vi "ContextHelp_PopUp.vi"() -> ()   [LabVIEW 2020]
uses:
  <resource>/Framework/Providers/Open_GDS/UML/ContextHelp/ContextHelp_EventType.ctl
  <resource>/Framework/Providers/Open_GDS/UML/ContextHelp/ContextHelp_ShowType.ctl
  <vilib>/event_ctls.llb/eventvkey.ctl
panel:
  in  "CallerRef":refnum<vi>
  in  "OccSync":refnum<k4>
  in  "Event":T1
  out "new picture":picture
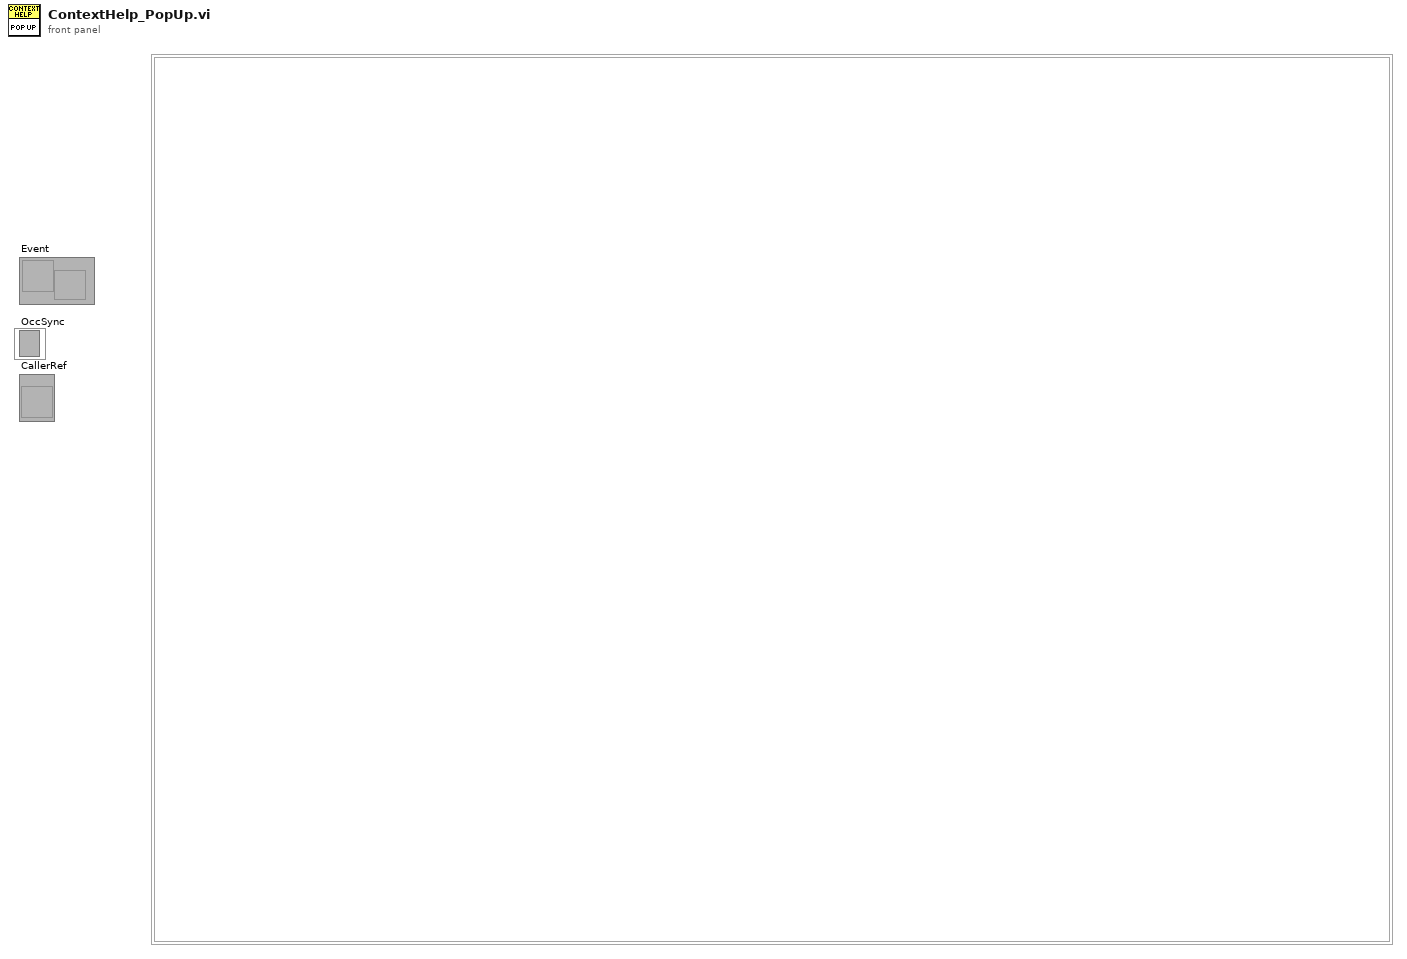
[diagram p1: front panel]
types:
  T1 = typedef "ContextHelp_EventType.ctl" = refnum<user-event>
  T2 = typedef "ContextHelp_ShowType.ctl" = cluster{"Header":string, "Picture":picture, "Text":string}
  T3 = cluster{"VIs":refnum<vi>[], "ViPathes":path[], "VI":i32, "Show":T2, "Win":cluster{"left":i16, "top":i16, "right":i16, "bottom":i16}, "LastViRef":refnum<vi>}
  T4 = enum32{"Custom", "Standard", "Using Panel", "Using SubVI", "Complete"}
  T5 = enum16{"SetPopUpEventTask", "GetStatus", "SetOpenState"}
  T6 = cluster{"left":i16, "top":i16, "right":i16, "bottom":i16}
  T7 = typedef "eventvkey.ctl" = enum16{"ASCII", "Enter", "Return", "Shift", "Ctrl", "Alt", "Cmd", "Opt", "Caps", "NumLock", "Clear", "Break", "Up", "Down", "Left", "Right", "Insert", "Delete", "Home", "End", "PageUp", "PageDown", "Escape", "Help", "Pause", "ScrollLock", "F1", "F2", "F3", "F4", "F5", "F6", "F7", "F8", "F9", "F10", "F11", "F12", "F13", "F14", "F15", "F16", "F17", "F18", "F19", "F20", "F21", "F22", "F23", "F24", "Play", "VolumeUp", "VolumeDown", "Mute", "Two Byte Char"}
  T8 = typedef "Librarian File Info Out.ctl" = cluster{"creation date":u32, "last mod date":u32, "type":string, "creator":string, "LV version":i32, "size":i32, "top level":bool}
  T9 = typedef "imagedata.ctl" = cluster{"image type":i32, "image depth":i32, "image":u8[], "mask":u8[], "colors":u32[], "Rectangle":cluster{"left":i16, "top":i16, "right":i16, "bottom":i16}}
  T10 = cluster{"Font Name:":string, "Size":i16, "Strikeout?":bool, "Italic?":bool, "Underline?":bool, "Outline?":bool, "Shadow?":bool, "Bold?":bool}
  T11 = enum16{"User-specified Font", "Application Font", "System Font", "Dialog Font"}
  T12 = typedef "LVRectTypeDef.ctl" = cluster{"Left":i16, "Top":i16, "Right":i16, "Bottom":i16}
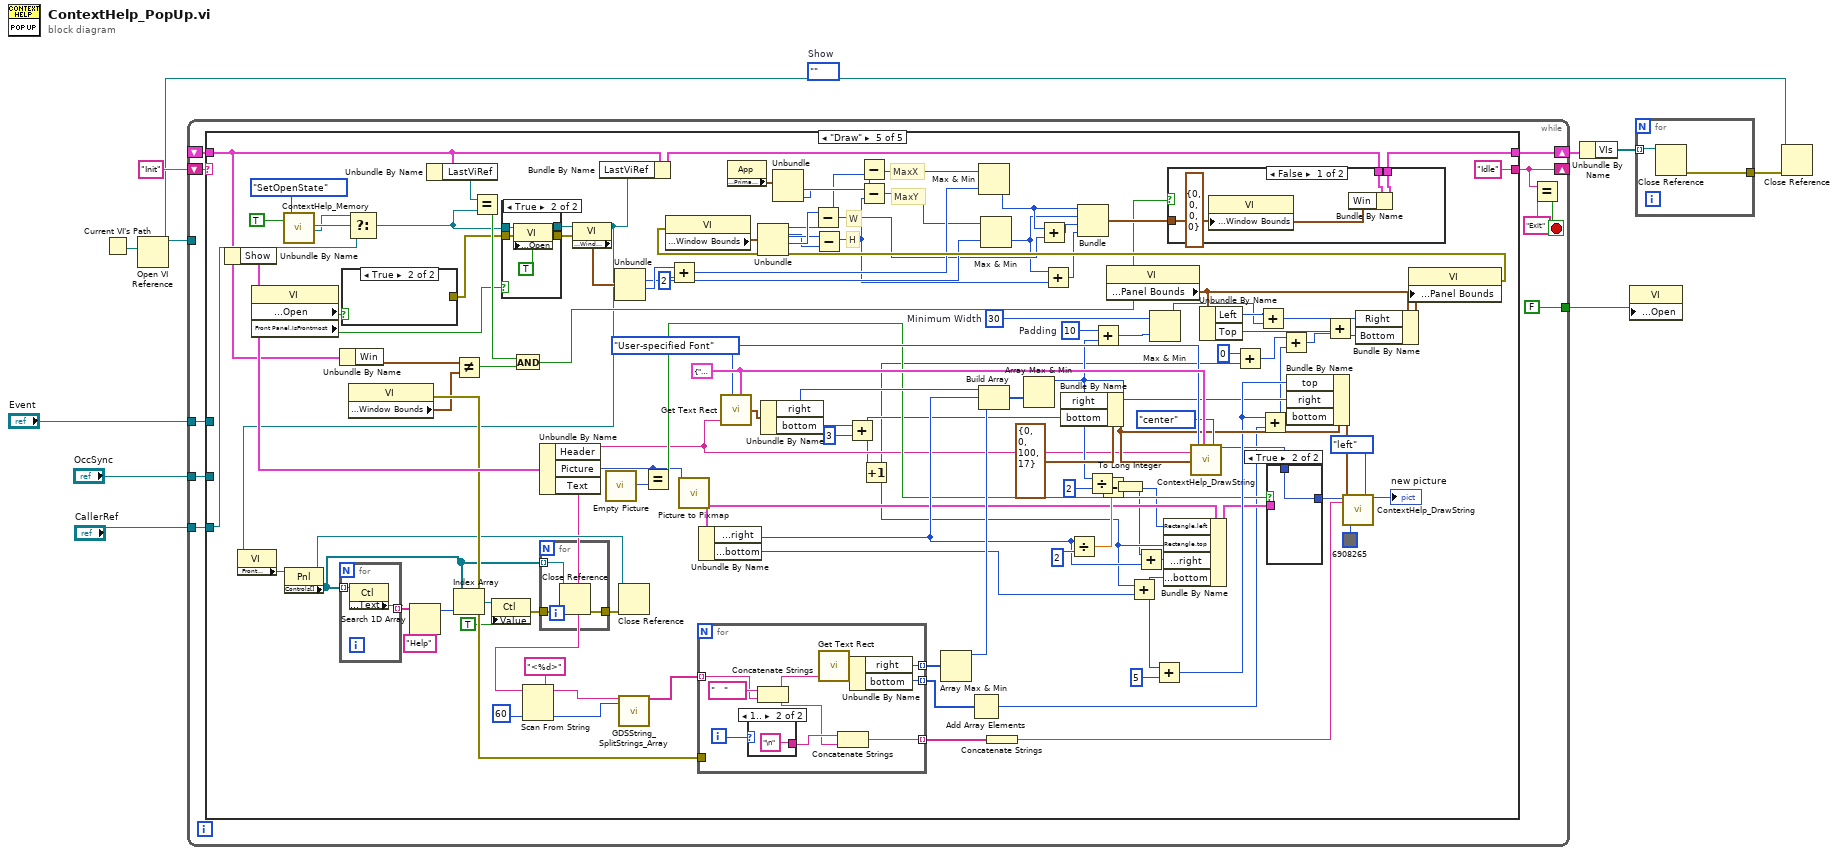
[diagram p0: block diagram]
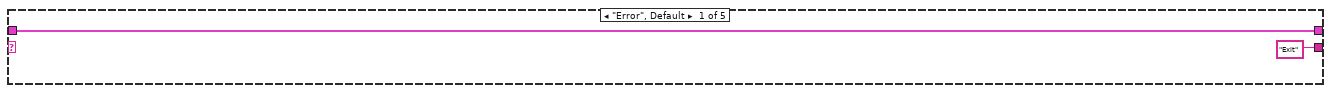
[diagram p2: hidden frame]
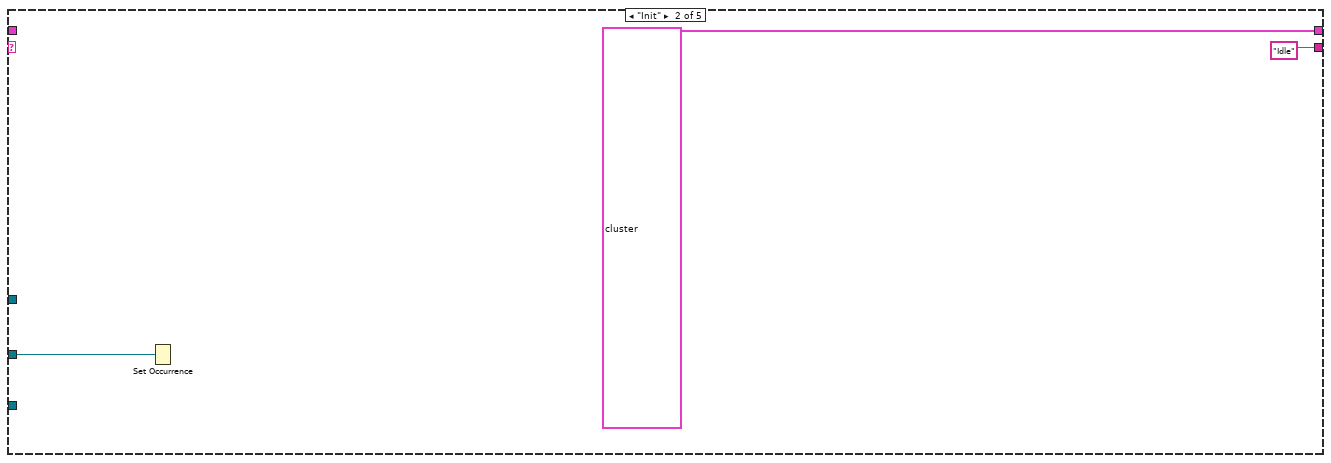
[diagram p3: hidden frame]
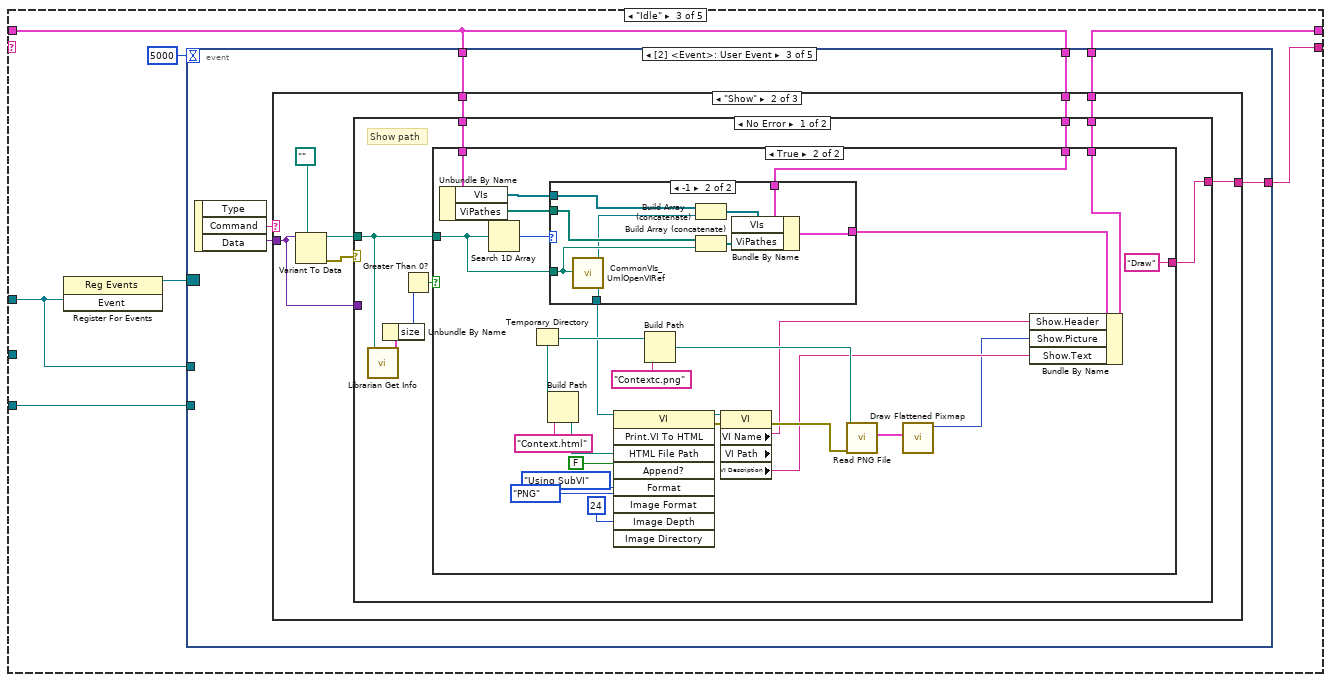
[diagram p4: hidden frame]
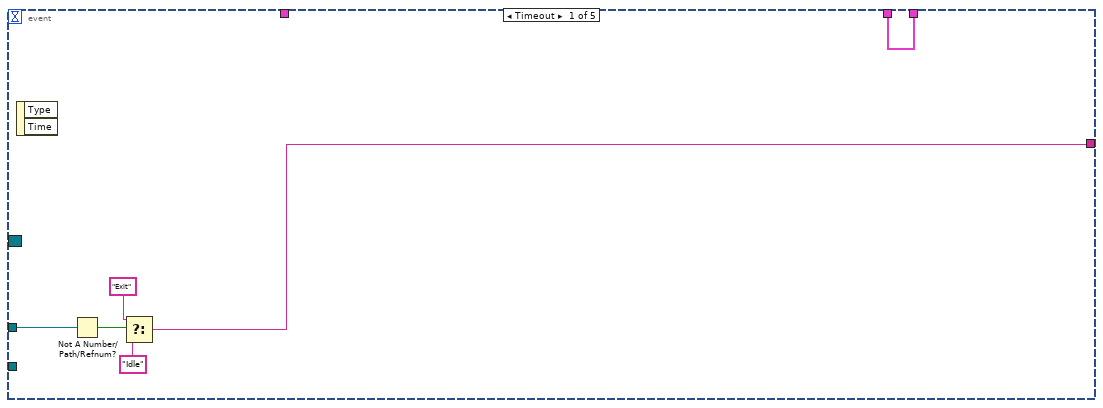
[diagram p5: hidden frame]
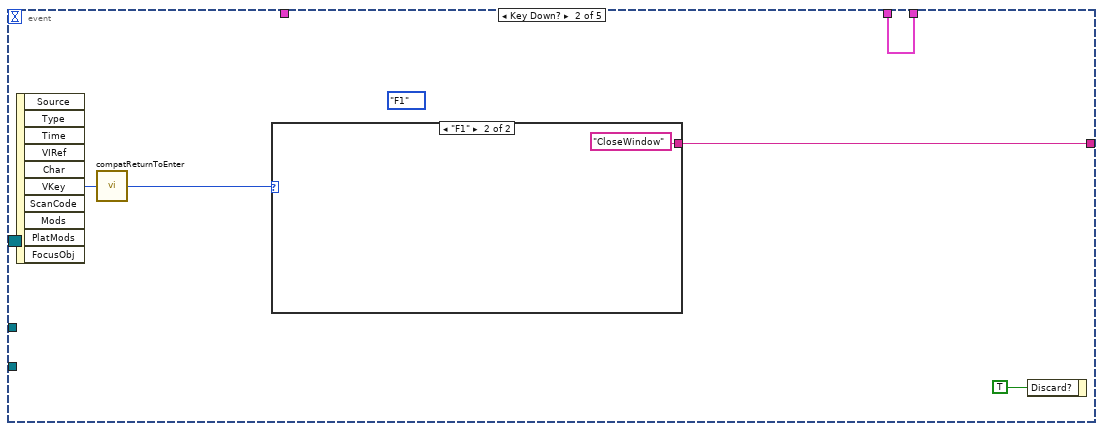
[diagram p6: hidden frame]
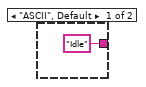
[diagram p7: hidden frame]
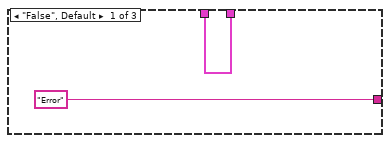
[diagram p8: hidden frame]
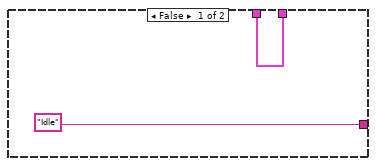
[diagram p9: hidden frame]
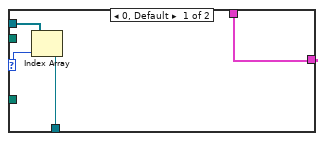
[diagram p10: hidden frame]
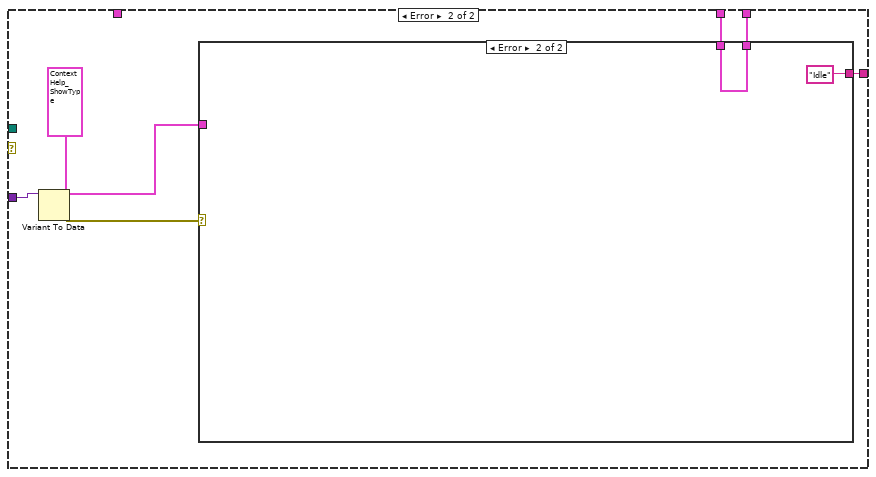
[diagram p11: hidden frame]
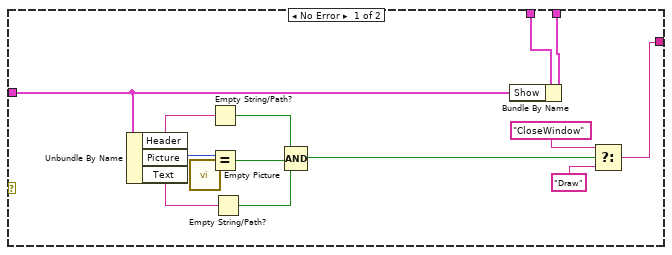
[diagram p12: hidden frame]
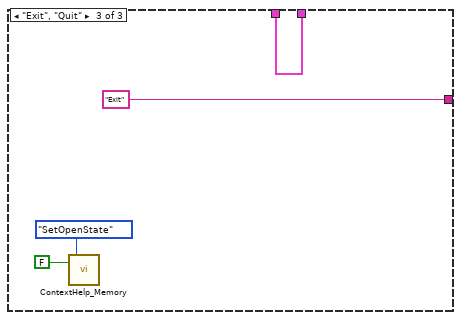
[diagram p13: hidden frame]
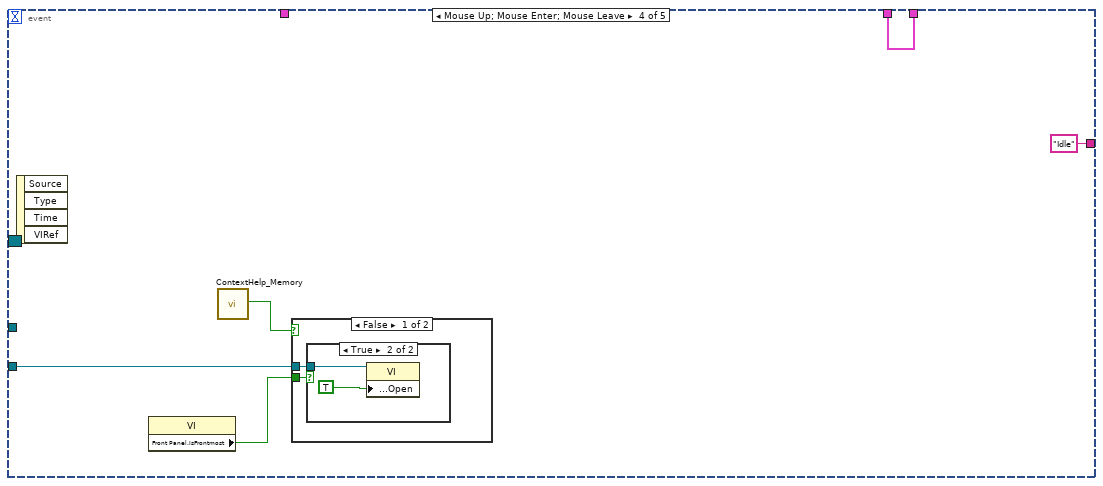
[diagram p14: hidden frame]
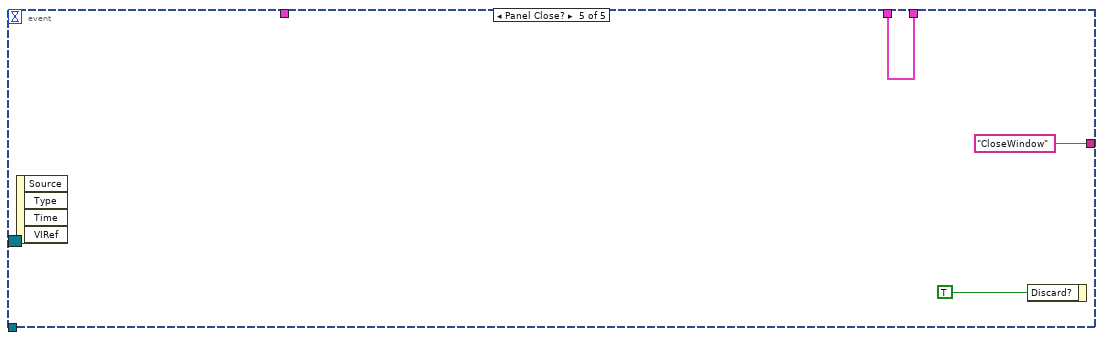
[diagram p17: hidden frame]
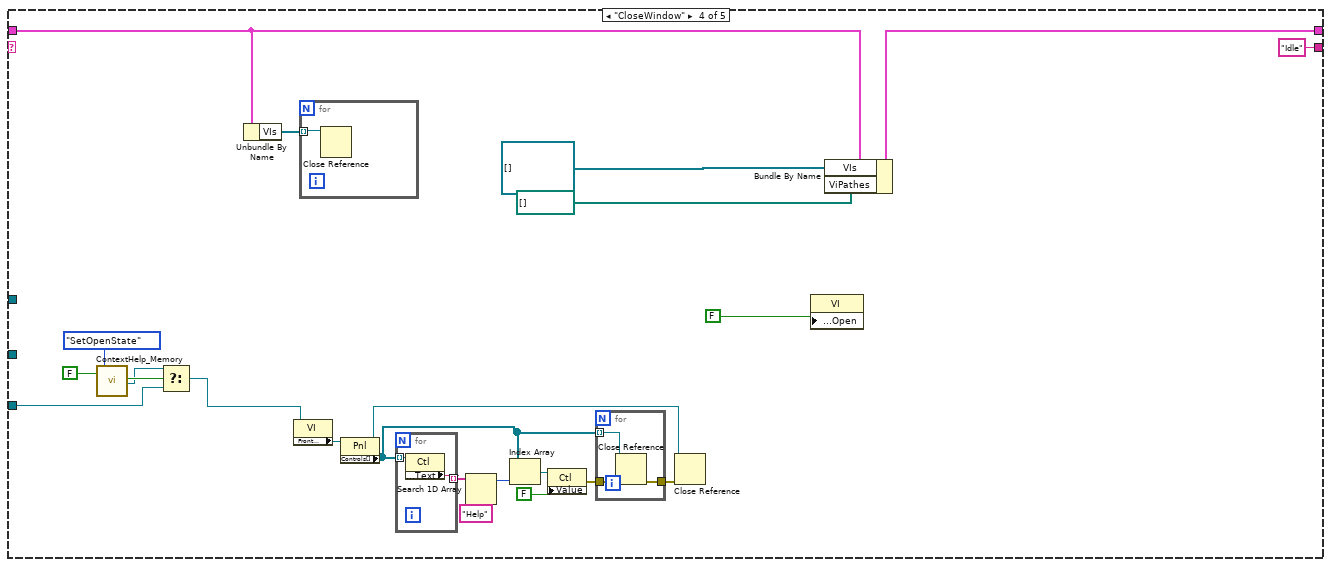
[diagram p18: hidden frame]
diagram:
  (unwired) enum16{"ClassDescription", ""}.""  # Show
  n1 = Current VI's Path() -> (path=w6:path)
  n2 = Open VI Reference(vi path=w6) -> (vi reference=w4:refnum<vi>)  [unwired: 2 in, 4 out]
  n3 = while {
    shift-right: [w19] -> _
    shift-left: "Init" -> [w20]
    shift-right: [w16] -> w8
    shift-left: _ -> [w15]
    tunnel: "Event" -> [w14]
    tunnel: w4 -> [_]
    tunnel: "OccSync" -> [w13]
    tunnel: [FALSE ("Front Panel Window:Open")] -> w2
    tunnel: "CallerRef" -> [w11]
    stop <- w17 stop-if-true
    n4 = case shown="\"Draw\"" w20 {
      tunnel: ["Exit" "Idle" w31 "Idle" "Idle"] -> w19
      tunnel: [w21 T3 {"VIs"=[], "ViPathes"=[], "VI"=0, "Show"={"Header"="", "Picture"=bytes[0], "Text"=""}, "Win"={"left"=0, "top"=0, "right"=0, "bottom"=0}, "LastViRef"=refnum} w30 w156 w210] -> w16
      tunnel: w15 -> [w21 _ w29 w157 w208]
      tunnel: w14 -> [_ _ w27 _ _]
      tunnel: w13 -> [_ w23 _ _ _]
      tunnel: w11 -> [_ _ w26 w150 w236]
      frame "Error", Default {
      }
      frame "Init" {
        n5 = Set Occurrence(w23) -> ()
      }
      frame "Idle" {
        n6 = register-events(w27) -> (reference out=w32:refnum<event-registration>)  [unwired: 2 in, 1 out]
        n7 = event shown="[2] <Event>: User Event" {
          selector: w32 -> [_ _ _ _ _]
          dyn-events: _ -> [_ _ _ _ _]
          timeout: 5000 -> [_ _ _ _ _]
          tunnel: [w34 w41 w50 "Idle" "CloseWindow"] -> w31
          tunnel: w29 -> [w38 w43 w49 w141 w146]
          tunnel: [w38 w43 w48 w141 w146] -> w30
          tunnel: w29 -> [_ _ w46 _ _]
          tunnel: w27 -> [w37 _ _ _ _]
          tunnel: w26 -> [_ _ _ w139 _]
          event Timeout {
            n8 = event-data() -> ()  [unwired: 3 out]
            n9 = Not A Number/Path/Refnum?(number/path/refnum=w37) -> (NaN/Path/Refnum?=w36:bool)
            n10 = Select(t="Exit", s=w36, f="Idle") -> (s? t:f=w34:string)
          }
          event Key Down? {
            (unwired) eventvkey."F1" ("VKey")
            n11 = event-data() -> ("VKey"=w39:T7)  [unwired: 10 out]
            n12 = call <vilib>:"compatReturnToEnter.vi"("VKey"=w39) -> ("VKey"=w42:T7)
            n13 = case shown="\"F1\"" w42 {
              tunnel: ["Idle" "CloseWindow"] -> w41
              frame "ASCII", Default {
              }
              frame "F1" {
              }
            }
            n14 = event-data("Discard?"=TRUE) -> ()  [unwired: 1 in, 1 out]
          }
          event User Event {
            n15 = event-data() -> ("Command"=w51:string, "Data"=w47:variant)  [unwired: 2 out]
            n16 = case shown="\"Show\"" w51 {
              tunnel: ["Error" w56 "Exit"] -> w50
              tunnel: w49 -> [w53 w59 w135]
              tunnel: [w53 w58 w135] -> w48
              tunnel: w47 -> [_ w54 _]
              tunnel: w46 -> [_ w60 _]
              frame "False", Default {
              }
              frame "Show" {
                n17 = Variant To Data(type=path "", Variant=w54) -> (data=w57:path, error out=w55:errorcluster)  [unwired: 1 in]
                n18 = case shown="No Error" w55 {
                  tunnel: w60 -> [w69 _]
                  tunnel: w59 -> [w68 w115]
                  tunnel: [w67 w114] -> w58
                  tunnel: w57 -> [w65 _]
                  tunnel: [w66 w111] -> w56
                  tunnel: w54 -> [_ w116]
                  frame No Error {
                    # "Show path"
                    n19 = call <vilib>:"Librarian Get Info.vi"("path"=w65) -> ("file information"=w64:T8)  [unwired: 1 in, 9 out]
                    n20 = Unbundle By Name(w64) -> ("size"=w63:i32)
                    n21 = Greater Than 0?(x=w63) -> (x > 0?=w62:bool)
                    n22 = case shown="True" w62 {
                      tunnel: w69 -> [_ w97]
                      tunnel: w68 -> [w71 w95]
                      tunnel: [w71 w90] -> w67
                      tunnel: w65 -> [_ w92]
                      tunnel: ["Idle" "Draw"] -> w66
                      frame False {
                      }
                      frame True {
                        n23 = Unbundle By Name(w97) -> ("VIs"=w94:refnum<vi>[], "ViPathes"=w93:path[])
                        n24 = Search 1D Array(1D array=w93, element=w92) -> (index of element=w96:i32)  [unwired: 1 out]
                        n25 = Temporary Directory() -> (w81:path)
                        n26 = Build Path(base path=w81, name or relative path="Context.html") -> (appended path=w79:path)
                        n27 = case shown="-1" w96 {
                          selector: w96 -> [w101 _]
                          tunnel: w92 -> [_ w103]
                          tunnel: w95 -> [w98 w109]
                          tunnel: w94 -> [w100 w108]
                          tunnel: w93 -> [_ w105]
                          tunnel: [w98 w104] -> w89
                          tunnel: [w99 w102] -> w76
                          frame 0, Default {
                            n28 = Index Array(array=w100, index=w101) -> (element=w99:refnum<vi>)
                          }
                          frame -1 {
                            n29 = call <resource>:"CommonVIs_UmlOpenVIRef.vi"("ViPath/ViName"=w103) -> ("vi reference"=w102:refnum<vi>)  [unwired: 3 in, 7 out]
                            n30 = Build Array (concatenate)(w108, w102) -> (w107:refnum<vi>[])
                            n31 = Build Array (concatenate)(w105, w103) -> (w106:path[])
                            n32 = Bundle By Name(cluster=w109, "VIs"=w107, "ViPathes"=w106) -> (w104:T3)
                          }
                        }
                        n33 = invoke class="VI" method="Print.VI To HTML"(reference=w76, "HTML File Path"=w79, "Append?"=FALSE, "Format"=T4."Using SubVI", "Image Format"=enum32{"PNG", "JPEG", "GIF"}."PNG", "Image Depth"=24) -> (reference out=w86:refnum<vi>, error out=w85:errorcluster)  [unwired: 3 in, 7 out]
                        n34 = Build Path(base path=w81, name or relative path="Contextc.png" ("HTML File Path")) -> (appended path=w78:path)
                        n35 = property class="VI" props=["VI Name", "VI Path", "VI Description"](reference=w86, error in=w85) -> (error out=w84:errorcluster, "VI Name"=w75:string, "VI Description"=w74:string)  [unwired: 2 out]
                        n36 = call <vilib>:"Read PNG File.vi"("error in (no error)"=w84, "path to PNG file"=w78) -> ("image data"=w73:T9)  [unwired: 9 out]
                        n37 = call <vilib>:"Draw Flattened Pixmap.vi"("image data"=w73) -> ("new picture"=w72:picture)  [unwired: 1 in, 7 out]
                        n38 = Bundle By Name(cluster=w89, "Show.Header"=w75, "Show.Picture"=w72, "Show.Text"=w74) -> (w90:T3)
                      }
                    }
                  }
                  frame Error {
                    n39 = Variant To Data(type=T2 {"Header"="", "Picture"=bytes[0], "Text"=""} ("output cluster"), Variant=w116) -> (data=w113:T2, error out=w112:errorcluster)  [unwired: 1 in]
                    n40 = case shown="Error" w112 {
                      tunnel: w115 -> [w130 w131]
                      tunnel: [w129 w131] -> w114
                      tunnel: w113 -> [w128 _]
                      tunnel: [w119 "Idle"] -> w111
                      frame No Error {
                        n41 = Unbundle By Name(w128) -> ("Header"=w124:string, "Picture"=w127:picture, "Text"=w125:string)
                        n42 = call "Empty Picture"() -> ("empty picture"=w126:picture)
                        n43 = Empty String/Path?(string/path=w124) -> (empty?=w123:bool)
                        n44 = Equal?(x=w127, y=w126) -> (x = y?=w122:bool)
                        n45 = Empty String/Path?(string/path=w125) -> (empty?=w121:bool)
                        n46 = Compound Arithmetic op=AND(w123, w122, w121) -> (w117:bool)
                        n47 = Bundle By Name(cluster=w130, "Show"=w128) -> (w129:T3)
                        n48 = Select(t="CloseWindow", s=w117, f="Draw") -> (s? t:f=w119:string)
                      }
                      frame Error {
                      }
                    }
                  }
                }
              }
              frame "Exit", "Quit" {
                n49 = call <resource>:"ContextHelp_Memory.vi"("State"=FALSE ("OpenState"), "Actio(GetStatus)n"=T5."SetOpenState") -> ()  [unwired: 2 in, 16 out]
              }
            }
          }
          event Mouse Up; Mouse Enter; Mouse Leave {
            n50 = event-data() -> ()  [unwired: 5 out]
            n51 = property class="VI"() -> ("Front Panel.IsFrontmost"=w137:bool)  [unwired: 2 in, 2 out]
            n52 = call <resource>:"ContextHelp_Memory.vi"() -> ("DialogCaller"=w138:bool)  [unwired: 4 in, 15 out]
            n53 = case shown="False" w138 {
              tunnel: w139 -> [w143 _]
              tunnel: w137 -> [w142 _]
              frame False {
                n54 = case shown="True" w142 {
                  tunnel: w143 -> [_ w145]
                  frame False {
                  }
                  frame True {
                    n55 = property class="VI"(reference=w145, "Front Panel Window:Open"=TRUE ("Front Panel Window:Is Frontmost")) -> ()  [unwired: 1 in, 2 out]
                  }
                }
              }
              frame True {
              }
            }
          }
          event Panel Close? {
            n56 = event-data() -> ()  [unwired: 5 out]
            n57 = event-data("Discard?"=TRUE) -> ()  [unwired: 1 in, 1 out]
          }
        }
      }
      frame "CloseWindow" {
        n58 = call <resource>:"ContextHelp_Memory.vi"("State"=FALSE ("OpenState"), "Actio(GetStatus)n"=T5."SetOpenState") -> ("DialogCaller"=w152:bool, "DialogRef"=w151:refnum<vi>)  [unwired: 2 in, 14 out]
        n59 = Select(t=w151, s=w152, f=w150) -> (s? t:f=w149:refnum<vi>)
        n60 = Unbundle By Name(w157) -> ("VIs"=w170:refnum<vi>[])
        n61 = property class="VI"(reference=w149) -> ("Front Panel"=w167:refnum<vi>)  [unwired: 1 in, 2 out]
        n62 = for {
          tunnel: w170 -> [w177] mode=indexing
          n63 = Close Reference(reference=w177) -> ()  [unwired: 1 in, 1 out]
        }
        n64 = property class="Pnl"(reference=w167) -> (reference out=w158:refnum<vi>, "Controls[]"=w160:refnum<vi>[])  [unwired: 1 in, 1 out]
        n65 = for {
          tunnel: w160 -> [w176] mode=indexing
          tunnel: [w175] -> w166 mode=indexing
          n66 = property class="Ctl"(reference=w176) -> ("Label.Text"=w175:string)  [unwired: 1 in, 2 out]
        }
        n67 = Search 1D Array(1D array=w166, element="Help") -> (index of element=w164:i32)  [unwired: 1 out]
        n68 = Index Array(array=w160, index=w164) -> (element=w163:refnum<vi>)
        n69 = property class="Ctl"(reference=w163, "Value"=FALSE ("Discard?")) -> (error out=w161:errorcluster)  [unwired: 1 in, 1 out]
        n70 = for {
          tunnel: w161 -> [w174]
          tunnel: w160 -> [w173] mode=indexing
          tunnel: [w172] -> w159
          n71 = Close Reference(reference=w173, error in (no error)=w174) -> (error out=w172:errorcluster)
        }
        n72 = Close Reference(reference=w158, error in (no error)=w159) -> ()  [unwired: 1 out]
        n73 = property class="VI"("Front Panel Window:Open"=FALSE) -> ()  [unwired: 2 in, 2 out]
        n74 = Bundle By Name(cluster=w157, "VIs"=refnum<vi>[] [], "ViPathes"=path[] []) -> (w156:T3)
      }
      frame "Draw" {
        w178 = i16 30  # Minimum Width
        w292 = T10 {"Font Name:"="Ariel", "Size"=14, "Strikeout?"=FALSE, "Italic?"=FALSE, "Underline?"=FALSE, "Outline?"=FALSE, "Shadow?"=FALSE, "Bold?"=TRUE} ("[user-specified font]")
        w247 = i16 10  # Padding
        w291 = T11."User-specified Font" ("desired font(Application)")
        # "MaxX"
        # "MaxY"
        # "H"
        # "W"
        n75 = Unbundle By Name(w208) -> ("Show"=w256:T2)
        n76 = property class="VI"() -> ("Front Panel Window:Open"=w241:bool, "Front Panel.IsFrontmost"=w181:bool)  [unwired: 2 in, 2 out]
        n77 = call <resource>:"ContextHelp_Memory.vi"("State"=TRUE ("OpenState"), "Actio(GetStatus)n"=T5."SetOpenState") -> ("DialogCaller"=w237:bool, "DialogRef"=w235:refnum<vi>)  [unwired: 2 in, 14 out]
        n78 = Unbundle By Name(w208) -> ("Win"=w206:T6)
        n79 = case shown="True" w241 {
          tunnel: [w314 _] -> w184
          frame False {
            n80 = property class="VI"("Front Panel Window:Open"=TRUE) -> (error out=w314:errorcluster)  [unwired: 2 in, 1 out]
          }
          frame True {
          }
        }
        n81 = Select(t=w235, s=w237, f=w236) -> (s? t:f=w185:refnum<vi>)
        n82 = property class="VI"() -> (error out=w211:errorcluster, "Front Panel Window:Window Bounds"=w207:T12)  [unwired: 2 in, 1 out]
        n83 = Unbundle By Name(w208) -> ("LastViRef"=w205:refnum<vi>)
        n84 = Not Equal?(x=w206, y=w207) -> (x != y?=w204:bool)
        n85 = Equal?(x=w205, y=w185) -> (x = y?=w186:bool)
        n86 = case shown="True" w181 {
          tunnel: w185 -> [w299 w304]
          tunnel: w184 -> [w298 w303]
          tunnel: [w299 w302] -> w183
          tunnel: [w298 w301] -> w182
          frame False {
          }
          frame True {
            n87 = property class="VI"(reference=w304, error in=w303, "Front Panel Window:Open"=TRUE) -> (reference out=w302:refnum<vi>, error out=w301:errorcluster)
          }
        }
        n88 = And(x=w186, y=w204) -> (x .and. y?=w203:bool)
        n89 = Unbundle By Name(w256) -> ("Header"=w251:string, "Picture"=w253:picture, "Text"=w187:string)
        n90 = Scan From String(format string="<%d>" ("regular expression"), input string=w187, default 1=60 ("Max string length")) -> (remaining string=w188:string, output 1=w189:i32)  [unwired: 2 in, 2 out]
        n91 = property class="VI"(reference=w183, error in=w182) -> (reference out=w192:refnum<vi>, "Front Panel Window:Window Bounds"=w225:T12)  [unwired: 1 out]
        n92 = property class="VI"(reference=w192) -> ("Front Panel"=w202:refnum<vi>)  [unwired: 1 in, 2 out]
        n93 = property class="Pnl"(reference=w202) -> (reference out=w193:refnum<vi>, "Controls[]"=w195:refnum<vi>[])  [unwired: 1 in, 1 out]
        n94 = for {
          tunnel: w195 -> [w309] mode=indexing
          tunnel: [w308] -> w201 mode=indexing
          n95 = property class="Ctl"(reference=w309) -> ("Label.Text"=w308:string)  [unwired: 1 in, 2 out]
        }
        n96 = Search 1D Array(1D array=w201, element="Help") -> (index of element=w199:i32)  [unwired: 1 out]
        n97 = Index Array(array=w195, index=w199) -> (element=w198:refnum<vi>)
        n98 = property class="Ctl"(reference=w198, "Value"=TRUE ("Discard?")) -> (error out=w196:errorcluster)  [unwired: 1 in, 1 out]
        n99 = for {
          tunnel: w196 -> [w307]
          tunnel: w195 -> [w306] mode=indexing
          tunnel: [w305] -> w194
          n100 = Close Reference(reference=w306, error in (no error)=w307) -> (error out=w305:errorcluster)
        }
        n101 = Bundle By Name(cluster=w208, "LastViRef"=w192) -> (w209:T3)
        n102 = call "Empty Picture"() -> ("empty picture"=w255:picture)
        n103 = Unbundle(w225) -> ("Top"=w218:i16, "Right"=w224:i16)  [unwired: 2 out]
        n104 = Close Reference(reference=w193, error in (no error)=w194) -> ()  [unwired: 1 out]
        n105 = call <resource>:"GDSString_SplitStrings_Array.vi"("string"=w188, "Max string length"=w189) -> ("Array"=w259:string[])  [unwired: 17 out]
        n106 = Equal?(x=w253, y=w255) -> (x = y?=w254:bool)
        n107 = Add(x=w224, y=i16 2) -> (x+y=w220:i16)
        n108 = call <vilib>:"Picture to Pixmap.vi"("picture"=w253) -> ("image data"=w252:T9)  [unwired: 3 in, 7 out]
        n109 = for {
          tunnel: w259 -> [w324] mode=indexing
          tunnel: [w327] -> w296 mode=indexing
          tunnel: [w326] -> w243 mode=indexing
          tunnel: [w323] -> w258 mode=indexing
          tunnel: w211 -> [_]
          i -> [w322]
          n110 = case shown="1.." w322 {
            tunnel: ["" "\n"] -> w321
            frame 0, Default {
            }
            frame 1.. {
            }
          }
          n111 = Concatenate Strings("   " ("replace string (\"\")"), w324) -> (w320:string)
          n112 = call <vilib>:"Get Text Rect.vi"("text"=w320) -> ("rect"=w328:T6)  [unwired: 5 in, 3 out]
          n113 = Concatenate Strings(w321, w320) -> (w323:string)
          n114 = Unbundle By Name(w328) -> ("right"=w327:i16, "bottom"=w326:i16)
        }
        n115 = Unbundle By Name(w252) -> ("Rectangle.right"=w281:i16, "Rectangle.bottom"=w282:i16)
        n116 = call <vilib>:"Get Text Rect.vi"("desired font(Application)"=w291, "text"=w251, "[user-specified font]"=w292) -> ("rect"=w297:T6)  [unwired: 3 in, 3 out]
        n117 = property class="App"() -> ("Display:Primary Workspace"=w228:T12)  [unwired: 2 in, 2 out]
        n118 = Unbundle By Name(w297) -> ("right"=w295:i16, "bottom"=w250:i16)
        n119 = Unbundle(w228) -> ("Right"=w227:i16, "Bottom"=w226:i16)  [unwired: 2 out]
        n120 = Add(x=w250, y=i16 3) -> (x+y=w248:i16)
        n121 = Increment(x=w248) -> (x+1=w244:i16)
        n122 = Array Max & Min(array=w296) -> (max value=w294:i16)  [unwired: 3 out]
        n123 = Add Array Elements(numeric array=w243) -> (sum=w242:i16)
        n124 = Build Array(w295, w281, w294) -> (w293:i16[])
        n125 = Concatenate Strings(w258) -> (w257:string)
        n126 = Array Max & Min(array=w293) -> (max value=w267:i16)  [unwired: 3 out]
        n127 = Bundle By Name(cluster=T6 {"left"=0, "top"=0, "right"=100, "bottom"=17} ("rect"), "right"=w267, "bottom"=w248) -> (w276:T6)
        n128 = Divide(x=w281, y=i16 2) -> (x/y=w285:dbl)
        n129 = Divide(x=w267, y=i16 2) -> (x/y=w287:dbl)
        n130 = Add(x=w247, y=w267) -> (x+y=w180:i16)
        n131 = Subtract(x=w287, y=w285) -> (x-y=w284:dbl)
        n132 = property class="VI"() -> ("Front Panel Window:Panel Bounds"=w269:T12)  [unwired: 2 in, 2 out]
        n133 = To Long Integer(number=w284) -> (32bit integer=w238:i32)
        n134 = Add(x=w244, y=w282) -> (x+y=w275:i16)
        n135 = Add(x=w238, y=w281) -> (x+y=w283:i32)
        n136 = Max & Min(x=w178, y=w180) -> (max(x,y)=w179:i16)  [unwired: 1 out]
        n137 = Add(x=w275, y=i16 5) -> (x+y=w273:i16)
        n138 = Bundle By Name(cluster=w252, "Rectangle.left"=w238, "Rectangle.top"=w244, "Rectangle.right"=w283, "Rectangle.bottom"=w275) -> (w271:T9)
        n139 = call <resource>:"ContextHelp_DrawString.vi"("Text"=w251, "rect"=w276, "desired font(Application)"=w291, "[user-specified font]"=w292, "Justify(center)"=enum16{"left", "center", "right"}."center") -> ("PictureOut"=w260:picture)  [unwired: 8 in, 6 out]
        n140 = Unbundle By Name(w269) -> ("Left"=w268:i16, "Top"=w263:i16)
        n141 = Add(x=i16 0, y=w244) -> (x+y=w246:i16)
        n142 = Add(x=w268, y=w179) -> (x+y=w265:i16)
        n143 = Add(x=w273, y=w242) -> (x+y=w266:i16)
        n144 = case shown="True" w254 {
          tunnel: [w318 w319] -> w280
          tunnel: w271 -> [w317 _]
          tunnel: w260 -> [w316 w319]
          frame False {
            n145 = call <vilib>:"Draw Flattened Pixmap.vi"("image data"=w317, "picture"=w316) -> ("new picture"=w318:picture)  [unwired: 7 out]
          }
          frame True {
          }
        }
        n146 = Add(x=w246, y=w266) -> (x+y=w262:i16)
        n147 = Bundle By Name(cluster=w276, "top"=w273, "right"=w267, "bottom"=w266) -> (w272:T6)
        n148 = Add(x=w263, y=w262) -> (x+y=w261:i16)
        n149 = call <resource>:"ContextHelp_DrawString.vi"("PictureIn"=w280, "Text"=w257, "rect"=w272, "text color(black)"=u32 6908265, "Justify(center)"=enum16{"left", "center", "right"}."left") -> ("PictureOut"=→"new picture":picture)  [unwired: 8 in, 6 out]
        n150 = Bundle By Name(cluster=w269, "Right"=w265, "Bottom"=w261) -> (w270:T12)
        n151 = property class="VI"("Front Panel Window:Panel Bounds"=w270) -> (error out=w234:errorcluster)  [unwired: 2 in, 1 out]
        n152 = property class="VI"(error in=w234) -> ("Front Panel Window:Window Bounds"=w233:T12)  [unwired: 1 in, 2 out]
        n153 = Unbundle(w233) -> ("Left"=w231:i16, "Top"=w229:i16, "Right"=w232:i16, "Bottom"=w230:i16)
        n154 = Subtract(x=w232, y=w231) -> (x-y=w215:i16)
        n155 = Subtract(x=w230, y=w229) -> (x-y=w212:i16)
        n156 = Subtract(x=w227, y=w215) -> (x-y=w221:i16)
        n157 = Subtract(x=w226, y=w212) -> (x-y=w219:i16)
        n158 = Max & Min(x=w221, y=w220) -> (min(x,y)=w217:i16)  [unwired: 1 out]
        n159 = Max & Min(x=w219, y=w218) -> (min(x,y)=w214:i16)  [unwired: 1 out]
        n160 = Add(x=w217, y=w215) -> (x+y=w216:i16)
        n161 = Add(x=w214, y=w212) -> (x+y=w213:i16)
        n162 = Bundle(w217, w214, w216, w213) -> (w222:cluster{i16, i16, i16, i16})  [unwired: 1 out]
        n163 = case shown="False" w203 {
          tunnel: w222 -> [w310 _]
          tunnel: w209 -> [w312 w313]
          tunnel: [w311 w313] -> w210
          frame False {
            (unwired) T6 {"left"=0, "top"=0, "right"=0, "bottom"=0} ("Front Panel Window:Window Bounds")
            n164 = property class="VI"("Front Panel Window:Window Bounds"=w310) -> ()  [unwired: 2 in, 2 out]
            n165 = Bundle By Name(cluster=w312, "Win"=w310) -> (w311:T3)
          }
          frame True {
          }
        }
      }
    }
    n166 = Equal?(x=w19, y="Exit") -> (x = y?=w17:bool)
  }
  n167 = Unbundle By Name(w8) -> ("VIs"=w7:refnum<vi>[])
  n168 = property class="VI"("Front Panel Window:Open"=w2) -> ()  [unwired: 2 in, 2 out]
  n169 = for {
    tunnel: w7 -> [w332] mode=indexing
    tunnel: [w331] -> w5
    n170 = Close Reference(reference=w332) -> (error out=w331:errorcluster)  [unwired: 1 in]
  }
  n171 = Close Reference(reference=w4, error in (no error)=w5) -> ()  [unwired: 1 out]
